vi "PicoScope2000aExampleEts.vi"() -> ()   [LabVIEW 2010]
uses:
  shared/PicoBuffers.ctl
  shared/Buffer and Transfer Settings.ctl
  shared/Acquisition Settings.ctl
  PicoScope2000aLib/PicoScope2000aAnalogChannelSettings.ctl
panel:
  in  "Trigger Settings":T1={"Trigger Enabled"=TRUE, "Trigger Source"=enum."Channel A", "Trigger Threshold (Volts)"=0.0, "Trigger Direction"=2, "Trigger Delay (samples)"=0, "Auto Trigger Time (ms)"=1000} {"Trigger Direction" items=["Rising"=2, "Falling"=3]}
  out "Device Info":T2
  in  "Channel A Settings":T3={"Enabled"=TRUE, "Coupling"=1, "Range"=6, "Analogue Offset"=0.0} {"Analogue Offset" format="%#_6p"; "Range" items=["20 mV"=1, "50 mV"=2, "100 mV"=3, "200 mV"=4, "500 mV"=5, "1 V"=6, "2 V"=7, "5 V"=8, "10 V"=9, "20 V"=10]; "Coupling" items=["AC", "DC"]}
  out "Properties Panel":T4 {"Max Total Capture Time Available (sec)" format="%.3p"; "Sample Frequency" format="%.3p"; "Sample Rate" format="%.3p"; "Max Samples Available" format="%.3p"; "Total Capture Time (sec)" format="%.3p"}
  out "EtsTimeValues":i64[](array[numeric])
  in  "etsInterleave":i16=10
  in  "etsCycles":i16=100
  in  "ETS Mode":u32(ring)=1 items=["PS2000A_ETS_OFF", "PS2000A_ETS_FAST", "PS2000A_ETS_SLOW"]
  out "overflow":i16 format="%06b"
  in  "Apply Settings":bool
  out "error out":errorcluster
  in  "Data file":path=path "PicoScope2000aExampleETS ChA Data"
  in  "Buffer and Transfer Settings":T5={"startIndex"=0, "Samples"=1000, "Down Sample Ratio"=1, "Down-Sample Mode"=0} {"Down-Sample Mode" items=["RAW none"=2147483648, "None"=0, "Aggregate"=1, "Decimate"=2, "Average"=4]; "Down Sample Ratio" step=1; "Samples" format="%_6p"}
  in  "Acquisition Settings":T6={"preTriggerSamples"=0, "postTriggerSamples"=1000, "timebase"=0} {"postTriggerSamples" format="%_6p"; "preTriggerSamples" format="%_6p"}
  in  "stop":bool
  out "Channel A":cluster{i32, sgl, "Data":dbl[]}(graph)
  in  "Serial Number":string
  in  "Use Serial Number":bool
  in  "error in (no error)":errorcluster
  # "Bit 0 = ChA"
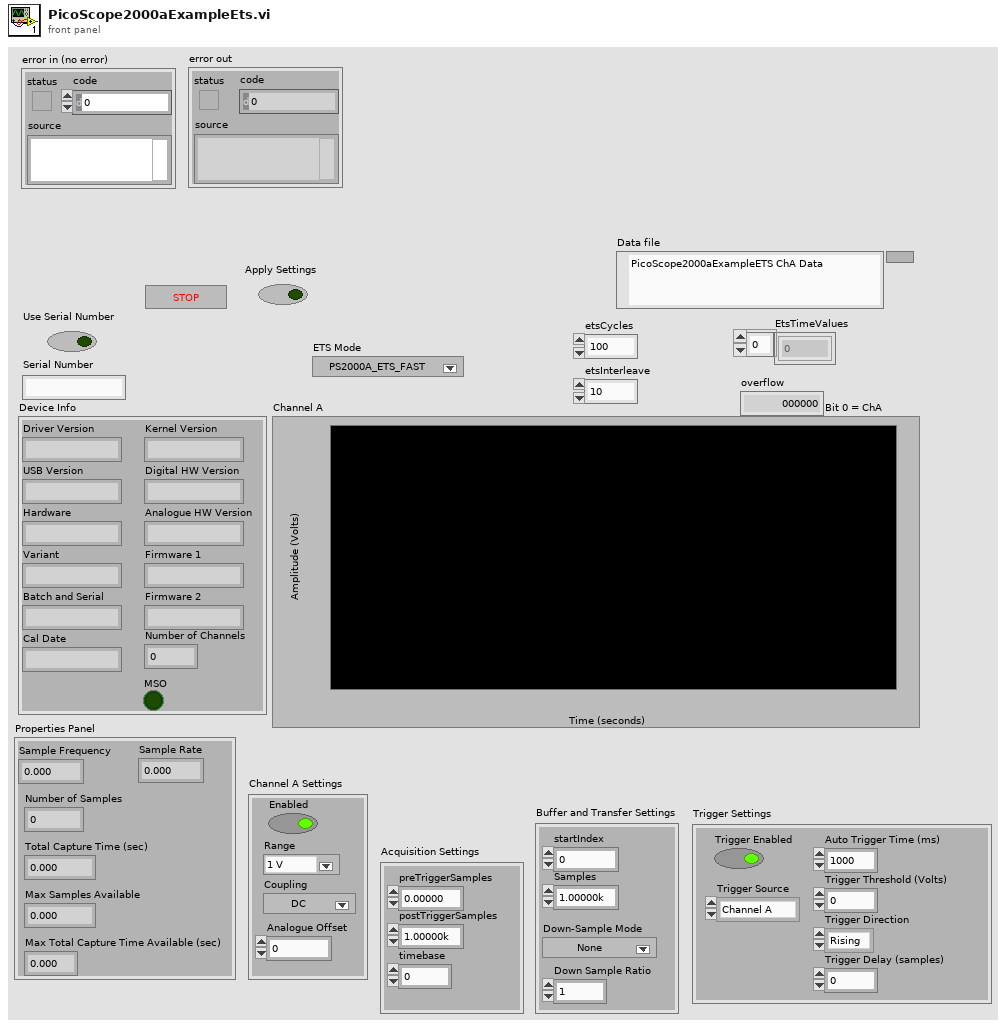
[diagram p1: front panel]
types:
  T1 = cluster{"Trigger Enabled":bool, "Trigger Source":enum16{"Channel A", "Channel B", "Channel C", "Channel D", "Ext."}, "Trigger Threshold (Volts)":dbl, "Trigger Direction":u16, "Trigger Delay (samples)":u32, "Auto Trigger Time (ms)":i16}
  T2 = cluster{"Driver Version":string, "USB Version":string, "Hardware":string, "Variant":string, "Batch and Serial":string, "Cal Date":string, "Kernel Version":string, "Digital HW Version":string, "Analogue HW Version":string, "Firmware 1":string, "Firmware 2":string, "MSO":bool, "Number of Channels":i16}
  T3 = typedef "PicoScope2000aAnalogChannelSettings.ctl" = cluster{"Enabled":bool, "Coupling":i16, "Range":u16, "Analogue Offset":sgl}
  T4 = cluster{"Sample Frequency":sgl, "Sample Rate":sgl, "Max Samples Available":i32, "Number of Samples":u32, "Total Capture Time (sec) ":sgl, "Max Total Capture Time Available (sec)":sgl}
  T5 = typedef "Buffer and Transfer Settings.ctl" = cluster{"startIndex":u64, "Samples":u64, "Down Sample Ratio":u64, "Down-Sample Mode":u32}
  T6 = typedef "Acquisition Settings.ctl" = cluster{"preTriggerSamples":u64, "postTriggerSamples":u64, "timebase":u32}
  T7 = enum16{"open", "open or create", "create or replace", "create", "open (read-only)"}
  T8 = typedef "PicoBuffers.ctl" = cluster{"Max Buffer Pointers":u64[][][], "Min Buffer Pointers":u64[][][], "StreamingDataInfo":cluster{"Channel":u32, "Down-Sample Mode":u32, "PICO_DATA_TYPE":enum32{"PICO_INT8_T", "PICO_INT16_T", "PICO_INT32_T", "PICO_UINT32_T", "PICO_INT64_T", ""}, "Samples":i32, "bufferIndex":u64, "startIndex":i32, "overflow":i16}[][]}
  T9 = cluster{"Sample Frequency":sgl, "Sample Internal":sgl, "Max Samples Available":i32, "Number of Samples":u32, "Total Capture Time (sec) ":sgl, "Max Total Capture Time Available (sec)":sgl}
  T10 = cluster{"Channel A Buffer":i16[], "Channel B Buffer":i16[], "Channel C Buffer":i16[], "Channel D Buffer":i16[], "Channel E Buffer":i16[], "Channel F Buffer":i16[], "Channel G Buffer":i16[], "Channel H Buffer":i16[], "Port 0 Buffer":i16[], "Port 1 Buffer":i16[]}[]
  T11 = cluster{"Channel A Buffer":i16[], "Channel B Buffer":i16[], "Channel C Buffer":i16[], "Channel D Buffer":i16[], "Channel E Buffer":i16[], "Channel F Buffer":i16[], "Channel G Buffer":i16[], "Channel H Buffer":i16[], "Port 0 Buffer":i16[], "Port 1 Buffer":i16[]}
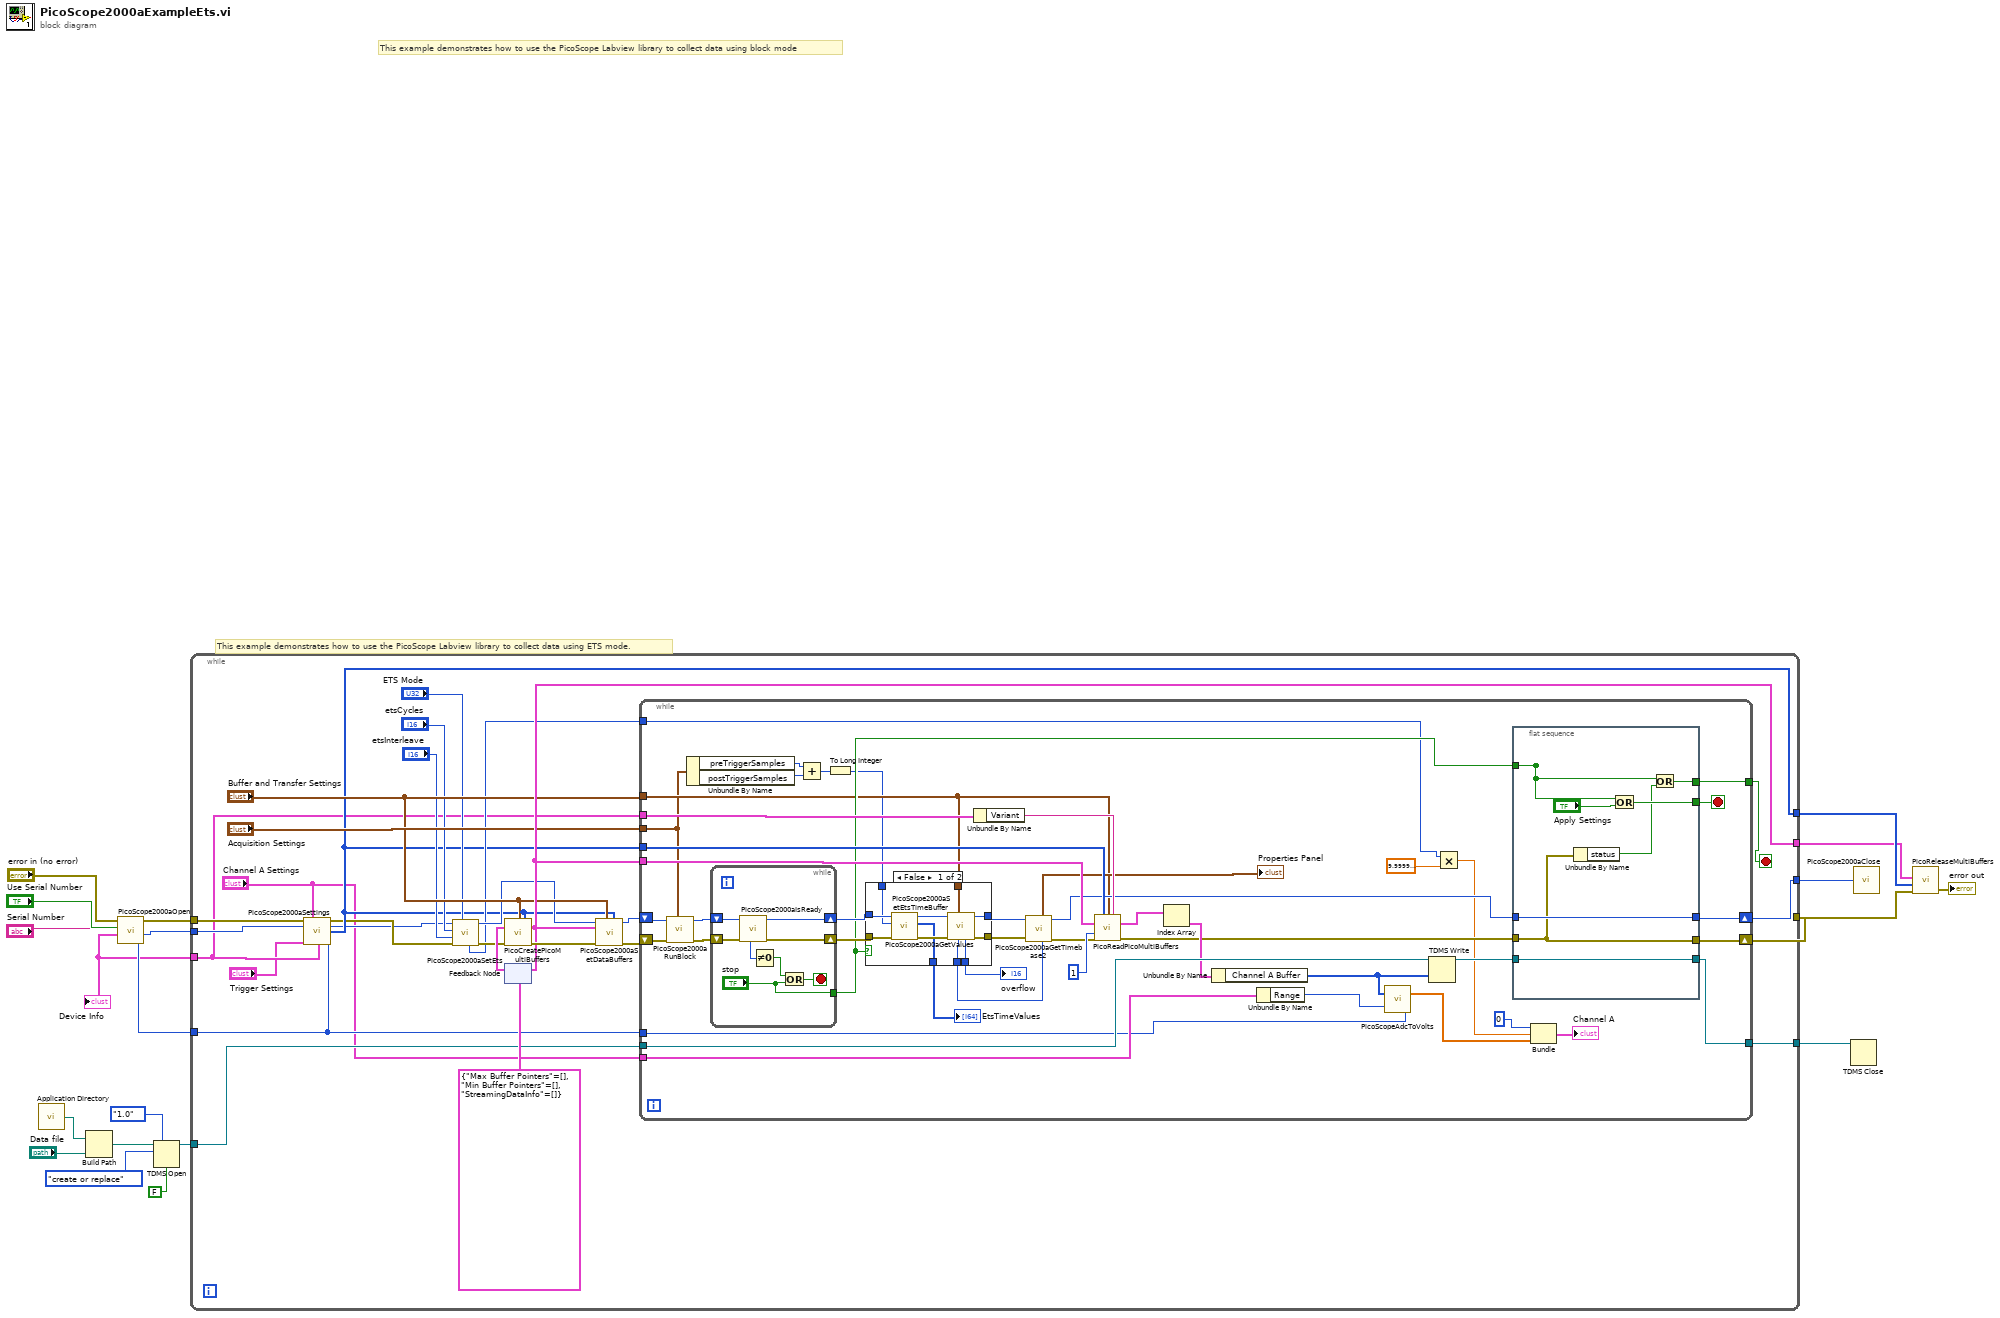
[diagram p0: block diagram]
diagram:
  # "This example demonstrates how to use the PicoScope Labview library to collect data using ETS mode."
  # "This example demonstrates how to use the PicoScope Labview library to collect data using block mode"
  n1 = call <vilib>:"Application Directory.vi"() -> ("Application Directory"=w12:path)
  n2 = Build Path(base path=w12, name or relative path="Data file") -> (appended path=w13:path)
  n3 = call "PicoScope2000aOpen.vi"("Serial Number"="Serial Number", "Use Serial Number"="Use Serial Number", "error in (no error)"="error in (no error)") -> ("Max Adc value"=w2:i16, "handle"=w20:i16, "error out"=w5:errorcluster, "Device Info"=w1:T2)  [unwired: 1 in]
  "Device Info" <- w1
  n4 = TDMS Open(6:FALSE ("disable buffering? (T)"), 7:enum16{"1.0", "2.0"}."1.0" ("file format version (2.0)"), 10:T7."create or replace" ("operation (0:open)"), 11:w13) -> (3:w10:refnum<k34>)  [unwired: 2 in, 1 out]
  n5 = while {
    tunnel: w20 -> [w23]
    tunnel: w2 -> [w26]
    tunnel: [w29] -> w19
    tunnel: [w45] -> w18
    tunnel: [w41] -> w11
    tunnel: w10 -> [w44]
    tunnel: w5 -> [w24]
    tunnel: [w42] -> w4
    tunnel: [w39] -> w3
    tunnel: w1 -> [w22]
    stop <- w40 stop-if-true
    n6 = call "PicoScope2000aSettings.vi"("error in"=w24, "Channel A Settings"="Channel A Settings", "handle in"=w23, "Trigger Settings"="Trigger Settings", "Device Info"=w22, "Max_adc"=w26) -> ("error out"=w28:errorcluster, "handle out"=w27:i16, "Enabled Array"=w29:i16[])  [unwired: 7 in]
    n7 = call "PicoScope2000aSetEts.vi"("ETS Mode"="ETS Mode", "error in (no error)"=w28, "etsInterleave"="etsInterleave", "etsCycles"="etsCycles", "handle in"=w27) -> ("error out"=w35:errorcluster, "handle out"=w34:i16, "sampleTimePicoseconds"=w33:i32)  [unwired: 4 in]
    n8 = feedback #1(T8 {"Max Buffer Pointers"=[], "Min Buffer Pointers"=[], "StreamingDataInfo"=[]} ("Data Pointers")) -> (w47:T8)
    n9 = call "PicoCreatePicoMultiBuffers.vi"("Buffer and Transfer Settings"="Buffer and Transfer Settings", "enabled array"=w29, "Data Pointers In"=w47, "error in (no error)"=w35) -> ("Data Pointers"=w45:T8, "error out"=w46:errorcluster)  [unwired: 10 in]
    n10 = feedback-in #1(w45) -> ()
    n11 = call "PicoScope2000aSetDataBuffers.vi"("enabled array"=w29, "Buffer and Transfer Settings"="Buffer and Transfer Settings", "error in (no error)"=w46, "Data Pointers In"=w45, "handle in"=w34) -> ("error out"=w38:errorcluster, "handle out"=w37:i16)  [unwired: 5 in]
    n12 = while {
      tunnel: w45 -> [w94]
      tunnel: "Buffer and Transfer Settings" -> [w60]
      tunnel: w29 -> [w89]
      tunnel: "Channel A Settings" -> [w88]
      tunnel: "Acquisition Settings" -> [w53]
      tunnel: w26 -> [w87]
      tunnel: w22 -> [w85]
      tunnel: [w75] -> w40
      shift-right: [w79] -> w42
      shift-left: w38 -> [w69]
      shift-right: [w73] -> w39
      shift-left: w37 -> [w70]
      tunnel: w44 -> [w93]
      tunnel: [w77] -> w41
      tunnel: w33 -> [w57]
      stop <- w74 stop-if-true
      n13 = call "PicoScope2000aRunBlock.vi"("Acquisition Settings"=w53, "error in (no error)"=w69, "handle in"=w70) -> ("error out"=w91:errorcluster, "handle out"=w90:i16)  [unwired: 5 in, 2 out]
      n14 = Unbundle By Name(w53) -> ("preTriggerSamples"=w52:u64, "postTriggerSamples"=w51:u64)
      n15 = while {
        shift-right: [w122] -> w71
        shift-left: w91 -> [w123]
        shift-right: [w121] -> w72
        shift-left: w90 -> [w120]
        tunnel: ["stop"] -> w68
        stop <- w117 stop-if-true
        n16 = call "PicoScope2000aIsReady.vi"("error in (no error)"=w123, "handle in"=w120) -> ("error out"=w122:errorcluster, "handle out"=w121:i16, "ready"=w119:i16)  [unwired: 7 in]
        n17 = Not Equal To 0?(x=w119) -> (x != 0?=w118:bool)
        n18 = Or(x=w118, y="stop") -> (x .or. y?=w117:bool)
      }
      n19 = Add(x=w52, y=w51) -> (x+y=w50:u64)
      n20 = To Long Integer(number=w50) -> (32bit integer=w49:i32)
      n21 = case shown="False" w68 {
        tunnel: w71 -> [w100 w106]
        tunnel: w72 -> [w97 w107]
        tunnel: [w105 w107] -> w63
        tunnel: [w104 w106] -> w64
        tunnel: w60 -> [w103 _]
        tunnel: [w102 _] -> w67
        tunnel: [w101 _] -> w66
        tunnel: [w96 _] -> w56
        tunnel: w49 -> [w95 _]
        frame False {
          n22 = call "PicoScope2000aSetEtsTimeBuffer.vi"("error in (no error)"=w100, "bufferLth"=w95, "handle in"=w97) -> ("error out"=w99:errorcluster, "EtsTimeValues"=w96:i64[], "handle out"=w98:i16)  [unwired: 6 in]
          n23 = call "PicoScope2000aGetValues.vi"("Buffer and Transfer Settings"=w103, "error in (no error)"=w99, "handle in"=w98) -> ("error out"=w104:errorcluster, "handle out"=w105:i16, "overflow"=w102:i16, "noOfSamples"=w101:u64)  [unwired: 5 in]
        }
        frame True {
        }
      }
      "overflow" <- w67
      "EtsTimeValues" <- w56
      n24 = Unbundle By Name(w85) -> ("Variant"=w86:string)
      n25 = call "PicoScope2000aGetTimebase2.vi"("Number of Samples"=w66, "error in (no error)"=w64, "handle in"=w63) -> ("error out"=w62:errorcluster, "handle out"=w61:i16, "Properties Panel"=→"Properties Panel":T9)  [unwired: 6 in]
      n26 = call "PicoReadPicoMultiBuffers.vi"("enabled array"=w89, "Buffer and Transfer Settings"=w60, "Variant"=w86, "Data Pointers"=w94, "No of Buffers"=1, "error in (no error)"=w62) -> ("MultiBuffers (Max or non-aggregated)"=w92:T10, "error out"=w76:errorcluster)  [unwired: 7 in, 1 out]
      n27 = Index Array(array=w92) -> (element=w80:T11)  [unwired: 1 in]
      n28 = Unbundle By Name(w80) -> ("Channel A Buffer"=w81:i16[])
      n29 = Unbundle By Name(w88) -> ("Range"=w82:u16)
      n30 = call "PicoScopeAdcToVolts.vi"("Max_adc"=w87, "Range Index"=w82, "Data"=w81) -> ("Data"=w55:dbl[])
      n31 = TDMS Write(0:w93, 9:w81) -> (4:w78:refnum<k34>)  [unwired: 4 in, 3 out]
      n32 = Multiply(x=w57, y=sgl 1e-12) -> (x*y=w58:sgl)
      n33 = flat-sequence {
        tunnel: [w115] -> w74
        tunnel: [w108] -> _
        tunnel: [w112] -> w75
        tunnel: w61 -> [w111]
        tunnel: [w111] -> w73
        tunnel: w76 -> [w110]
        tunnel: [w110] -> w79
        tunnel: [w109] -> w77
        tunnel: w78 -> [w109]
        tunnel: w68 -> [w108]
        frame #0 {
          n34 = Unbundle By Name(w110) -> ("status"=w113:bool)
          n35 = Or(x=w108, y="Apply Settings") -> (x .or. y?=w115:bool)
          n36 = Or(x=w108, y=w113) -> (x .or. y?=w112:bool)
        }
      }
      n37 = Bundle(0, w58, "Data"=w55) -> (→"Channel A":cluster{i32, sgl, "Data":dbl[]})  [unwired: 1 in]
    }
  }
  n38 = TDMS Close(11:w11) -> ()  [unwired: 1 in, 2 out]
  n39 = call "PicoScope2000aClose.vi"("handle"=w3) -> ()
  n40 = call "PicoReleaseMultiBuffers.vi"("error in (no error)"=w4, "Enabled array"=w19, "Data Pointers"=w18) -> ("error out"=→"error out":errorcluster)  [unwired: 8 in]
